vi "DCW ini file Read.vi"(2 "configuration file path":path, 11 "error in (no error) 2":errorcluster) -> (3 "DWC Voltage":dbl, 4 "Ramp Time":dbl, 6 "DCW Test Time(S)":dbl, 8 "DCW LO SET":dbl, 10 "DCW HI SET":dbl, 15 "error in (no error) 3":errorcluster)   [LabVIEW 2021]
uses:
  Template/Main_VI/Control/Ini.ctl
panel:
  out "value":string
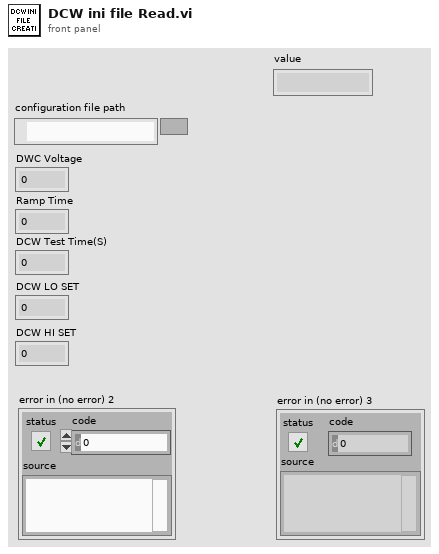
[diagram p1: front panel]
types:
  T1 = typedef "Ini.ctl" = enum16{"Write", "Read"}
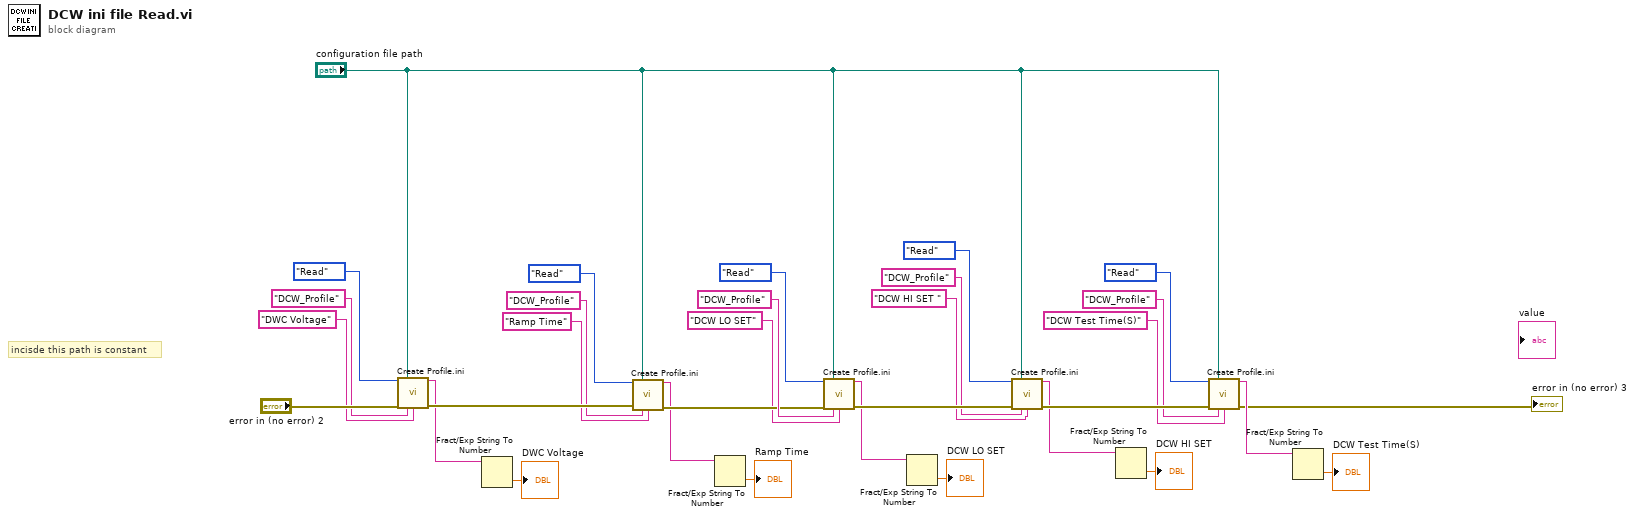
[diagram p0: block diagram]
diagram:
  # "incisde this path is constant"
  n1 = call "Create Profile.ini.vi"(0:Ini."Read", "configuration file path"="configuration file path", "error in (no error)"="error in (no error) 2", "Read Section"="DCW_Profile" ("Write Section"), "Read Key"="DWC Voltage" ("Write key")) -> ("value"=w12:string, "error in (no error) 3"=w27:errorcluster)  [unwired: 9 in]
  n2 = Fract/Exp String To Number(string=w12) -> (number=→"DWC Voltage":dbl)  [unwired: 3 in, 1 out]
  n3 = call "Create Profile.ini.vi"(0:Ini."Read", "configuration file path"="configuration file path", "error in (no error)"=w27, "Read Section"="DCW_Profile" ("Write Section"), "Read Key"="Ramp Time" ("Write key")) -> ("value"=w11:string, "error in (no error) 3"=w18:errorcluster)  [unwired: 9 in]
  n4 = Fract/Exp String To Number(string=w11) -> (number=→"Ramp Time":dbl)  [unwired: 3 in, 1 out]
  n5 = call "Create Profile.ini.vi"(0:Ini."Read", "configuration file path"="configuration file path", "error in (no error)"=w18, "Read Section"="DCW_Profile" ("Write Section"), "Read Key"="DCW LO SET" ("Write key")) -> ("value"=w10:string, "error in (no error) 3"=w26:errorcluster)  [unwired: 9 in]
  n6 = Fract/Exp String To Number(string=w10) -> (number=→"DCW LO SET":dbl)  [unwired: 3 in, 1 out]
  n7 = call "Create Profile.ini.vi"(0:Ini."Read", "configuration file path"="configuration file path", "error in (no error)"=w26, "Read Section"="DCW_Profile" ("Write Section"), "Read Key"="DCW HI SET " ("Write key")) -> ("value"=w9:string, "error in (no error) 3"=w25:errorcluster)  [unwired: 9 in]
  n8 = Fract/Exp String To Number(string=w9) -> (number=→"DCW HI SET":dbl)  [unwired: 3 in, 1 out]
  n9 = call "Create Profile.ini.vi"(0:Ini."Read", "configuration file path"="configuration file path", "error in (no error)"=w25, "Read Section"="DCW_Profile" ("Write Section"), "Read Key"="DCW Test Time(S)" ("Write key")) -> ("value"=w8:string, "error in (no error) 3"=→"error in (no error) 3":errorcluster)  [unwired: 9 in]
  n10 = Fract/Exp String To Number(string=w8) -> (number=→"DCW Test Time(S)":dbl)  [unwired: 3 in, 1 out]
